vi "Check Action.vi"(6 "HRS Time":dbl, 7 "Values In":dbl[](array[numeric]), 8 "error in (no error)":errorcluster, 11 "LatchedValve in":refnum<class "LatchedValve.lvclass">) -> (0 "error out":errorcluster, 2 "Actions":T1[](array[typedef]), 3 "LatchedValve out":refnum<class "LatchedValve.lvclass">, 5 "Values":dbl[](array[numeric]))   [LabVIEW 2020, in "VolatusControl.lvlib" / "LatchedValve.lvclass"]
uses:
  LatchedValve.lvclass
  Control Action.ctl
  LatchedValve.lvclass/LatchedValve.ctl
  State.ctl
  Volatus/MessageQ/MessageQ.lvclass
  VolatusControl.lvlib
  lv-vecto/Vecto/Vecto.lvlib
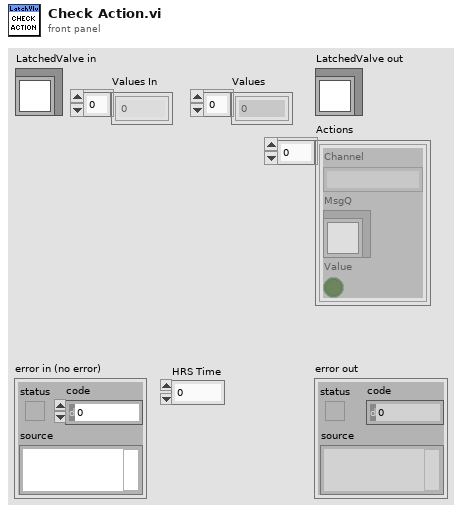
[diagram p1: front panel]
types:
  T1 = typedef "VolatusControl.lvlib/Control Action.ctl" = cluster{"Channel":string, "MsgQ":refnum<class "MessageQ.lvclass">, "Value":bool}
  T2 = typedef "VolatusControl.lvlib/LatchedValve.lvclass/State.ctl" = enum16{"Idle", "Cmd Dir", "Settle Dir", "Actuate", "Deactivate"}
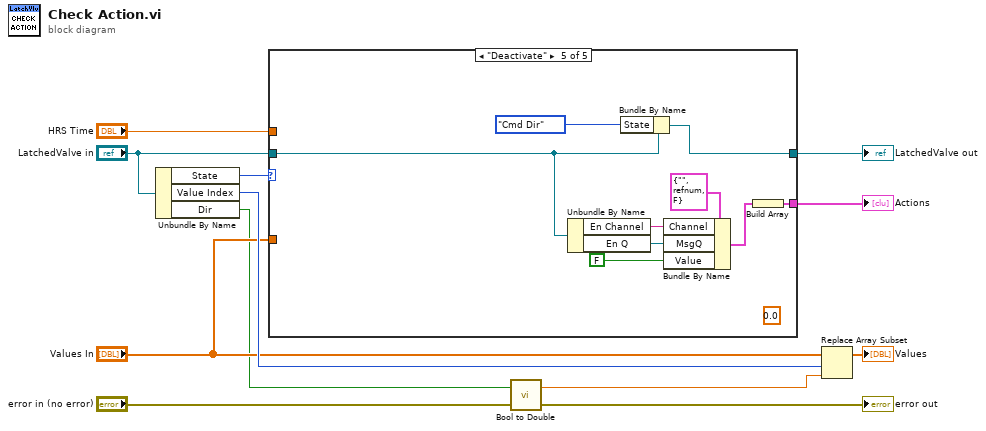
[diagram p0: block diagram]
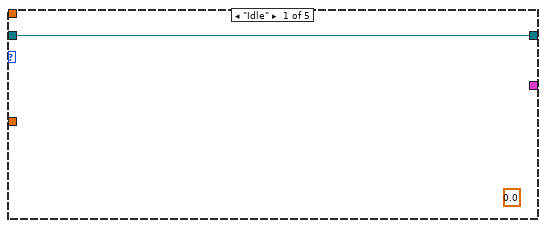
[diagram p2: hidden frame]
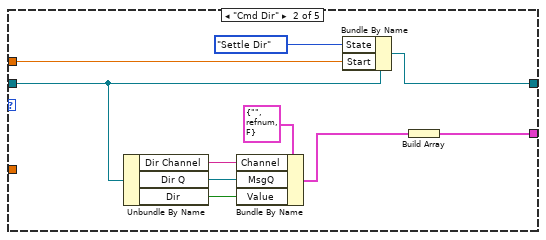
[diagram p3: hidden frame]
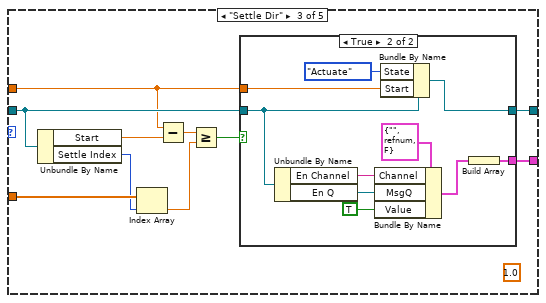
[diagram p4: hidden frame]
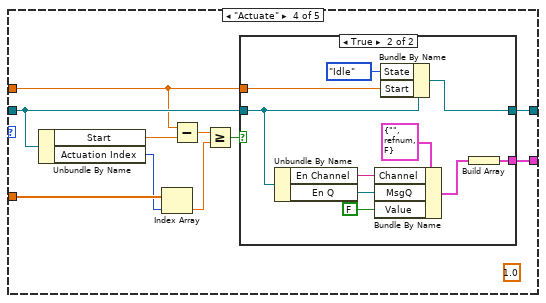
[diagram p6: hidden frame]
diagram:
  n1 = Unbundle By Name("LatchedValve in") -> ("State"=w10:T2, "Value Index"=w4:i32, "Dir"=w1:bool)
  n2 = case shown="\"Deactivate\"" w10 {
    tunnel: "LatchedValve in" -> [w12 w18 w29 w50 w67]
    tunnel: [w12 w17 w30 w51 w72] -> w9
    tunnel: [_ w13 w32 w53 w65] -> w8
    tunnel: "HRS Time" -> [_ w16 w28 w49 _]
    tunnel: "Values In" -> [_ _ w25 w46 _]
    frame "Idle" {
      (unwired) 0.0
    }
    frame "Cmd Dir" {
      n3 = Unbundle By Name(w18) -> ("Dir Channel"=w19:string, "Dir Q"=w20:refnum<class "MessageQ.lvclass">, "Dir"=w14:bool)
      n4 = Bundle By Name(cluster=T1 {"Channel"="", "MsgQ"=refnum, "Value"=FALSE} ("Action"), "Channel"=w19, "MsgQ"=w20, "Value"=w14) -> (w21:T1)
      n5 = Bundle By Name(cluster=w18, "State"=State."Settle Dir", "Start"=w16) -> (w17:refnum<class "LatchedValve.lvclass">)
      n6 = Build Array(w21) -> (w13:T1[])
    }
    frame "Settle Dir" {
      (unwired) 1.0
      n7 = Unbundle By Name(w29) -> ("Start"=w31:dbl, "Settle Index"=w24:i32)
      n8 = Index Array(array=w25, index=w24) -> (element=w23:dbl)
      n9 = Subtract(x=w28, y=w31) -> (x-y=w27:dbl)
      n10 = Greater Or Equal?(x=w27, y=w23) -> (x >= y?=w26:bool)
      n11 = case shown="True" w26 {
        tunnel: [_ w34] -> w32
        tunnel: [w33 w38] -> w30
        tunnel: w29 -> [w33 w37]
        tunnel: w28 -> [_ w35]
        frame False {
        }
        frame True {
          n12 = Unbundle By Name(w37) -> ("En Channel"=w40:string, "En Q"=w39:refnum<class "MessageQ.lvclass">)
          n13 = Bundle By Name(cluster=T1 {"Channel"="", "MsgQ"=refnum, "Value"=FALSE} ("Action"), "Channel"=w40, "MsgQ"=w39, "Value"=TRUE) -> (w42:T1)
          n14 = Bundle By Name(cluster=w37, "State"=State."Actuate", "Start"=w35) -> (w38:refnum<class "LatchedValve.lvclass">)
          n15 = Build Array(w42) -> (w34:T1[])
        }
      }
    }
    frame "Actuate" {
      (unwired) 1.0
      n16 = Unbundle By Name(w50) -> ("Start"=w52:dbl, "Actuation Index"=w45:i32)
      n17 = Index Array(array=w46, index=w45) -> (element=w44:dbl)
      n18 = Subtract(x=w49, y=w52) -> (x-y=w48:dbl)
      n19 = Greater Or Equal?(x=w48, y=w44) -> (x >= y?=w47:bool)
      n20 = case shown="True" w47 {
        tunnel: [_ w55] -> w53
        tunnel: [w54 w59] -> w51
        tunnel: w50 -> [w54 w58]
        tunnel: w49 -> [_ w56]
        frame False {
        }
        frame True {
          n21 = Unbundle By Name(w58) -> ("En Channel"=w61:string, "En Q"=w60:refnum<class "MessageQ.lvclass">)
          n22 = Bundle By Name(cluster=T1 {"Channel"="", "MsgQ"=refnum, "Value"=FALSE} ("Action"), "Channel"=w61, "MsgQ"=w60, "Value"=FALSE) -> (w63:T1)
          n23 = Bundle By Name(cluster=w58, "State"=State."Idle", "Start"=w56) -> (w59:refnum<class "LatchedValve.lvclass">)
          n24 = Build Array(w63) -> (w55:T1[])
        }
      }
    }
    frame "Deactivate" {
      (unwired) 0.0
      n25 = Unbundle By Name(w67) -> ("En Channel"=w69:string, "En Q"=w70:refnum<class "MessageQ.lvclass">)
      n26 = Bundle By Name(cluster=w67, "State"=State."Cmd Dir") -> (w72:refnum<class "LatchedValve.lvclass">)
      n27 = Bundle By Name(cluster=T1 {"Channel"="", "MsgQ"=refnum, "Value"=FALSE} ("Action"), "Channel"=w69, "MsgQ"=w70, "Value"=FALSE) -> (w68:T1)
      n28 = Build Array(w68) -> (w65:T1[])
    }
  }
  "LatchedValve out" <- w9
  "Actions" <- w8
  n29 = call "Bool to Double.vi"("Bool"=w1) -> ("Double"=w2:dbl)  [unwired: 2 in]
  n30 = Replace Array Subset(array="Values In", new element=w2, index=w4) -> (→"Values":dbl[])
  "error out" <- "error in (no error)"
